vi "Day 20.vi"() -> ()   [LabVIEW 2021]
uses:
  Day 20-Calculate Lookup Index.vi
  <vilib>/Utility/file.llb/Read Delimited Spreadsheet (string).vi
panel:
  out "Output Image":bool[][](array[boolean])
  out "Initial Image":bool[][](array[boolean])
  in  "Iterations":i32=50
  out "Count of \"Lit\"":u64
  in  "Input File":enum32{"example input", "input"}(radio)
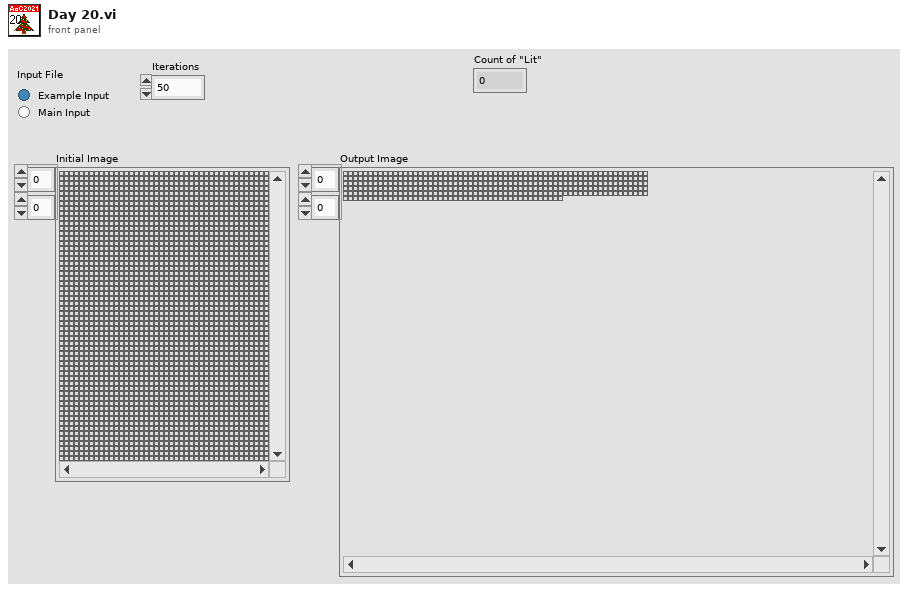
[diagram p1: front panel]
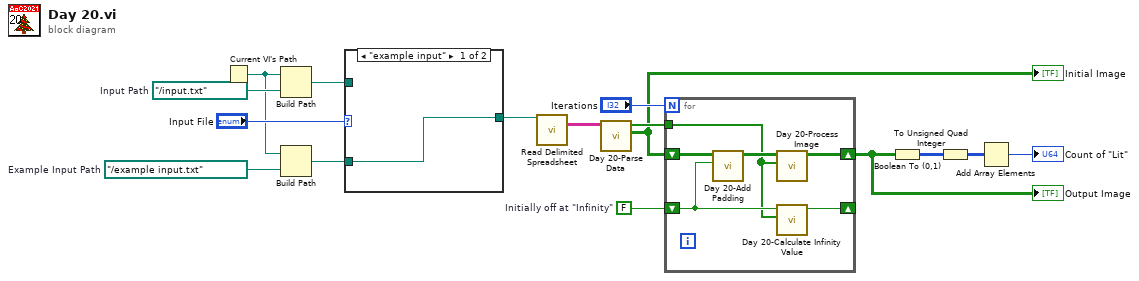
[diagram p0: block diagram]
diagram:
  w4 = FALSE  # Initially off at "Infinity"
  w15 = path "../example input.txt"  # Example Input Path
  w16 = path "../input.txt"  # Input Path
  n1 = Current VI's Path() -> (path=w10:path)
  n2 = Build Path(base path=w10, name or relative path=w16) -> (appended path=w13:path)
  n3 = Build Path(base path=w10, name or relative path=w15) -> (appended path=w12:path)
  n4 = case shown="\"example input\"" "Input File" {
    tunnel: w13 -> [_ w18]
    tunnel: w12 -> [w17 _]
    tunnel: [w17 w18] -> w11
    frame "example input" {
    }
    frame "input" {
    }
  }
  n5 = call-poly <vilib>:"Read Delimited Spreadsheet.vi"("file path (dialog if empty)"=w11) -> ("all rows"=w9:string[][])  [unwired: 9 in, 5 out]
  n6 = call "Day 20-Parse Data.vi"("Data in"=w9) -> ("Input Image"=w3:bool[][], "Image Enhancement Lookup"=w5:bool[])  [unwired: 9 in]
  "Initial Image" <- w3
  n7 = for {
    N: "Iterations" -> [_]
    tunnel: w5 -> [w19]
    shift-right: [w24] -> w2
    shift-left: w3 -> [w23]
    shift-right: [w20] -> _
    shift-left: w4 -> [w21]
    n8 = call "Day 20-Add Padding.vi"("Padding Value"=w21, "Array in"=w23) -> ("Array out"=w22:bool[][])  [unwired: 9 in]
    n9 = call "Day 20-Process Image.vi"("Lookup Array"=w19, "Image in"=w22) -> ("Image out"=w24:bool[][])  [unwired: 9 in]
    n10 = call "Day 20-Calculate Infinity Value.vi"("Lookup Array"=w19, "Previous \"Infinity\" Value"=w21) -> ("New \"Infinity\" Value"=w20:bool)  [unwired: 9 in]
  }
  "Output Image" <- w2
  n11 = Boolean To (0,1)(Boolean=w2) -> (0, 1=w8:i16[][])
  n12 = To Unsigned Quad Integer(1:w8) -> (0:w1:u64[][])
  n13 = Add Array Elements(numeric array=w1) -> (sum=→"Count of \"Lit\"":u64)
